vi "Init UI.vi"(8 "error in (no error)":errorcluster, 11 "HistorianCharting in":refnum<class "HistorianCharting.lvclass">) -> (0 "error out":errorcluster, 3 "HistorianCharting out":refnum<class "HistorianCharting.lvclass">)   [LabVIEW 2020, in "VolatusGUIElements.lvlib" / "HistorianCharting.lvclass"]
uses:
  HistorianCharting.lvclass
  HistorianCharting.lvclass/HistorianCharting.ctl
  <vilib>/dlg_ctls.llb/Space Constant.vi
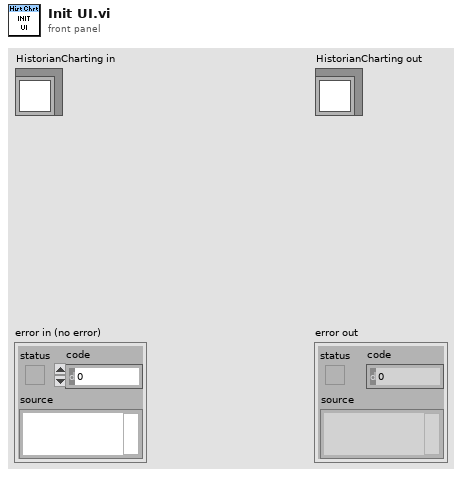
[diagram p1: front panel]
types:
  T1 = cluster{"Channel":string, "Value":dbl, "Color":u32, "Scale":bool, "Visible":bool}[]
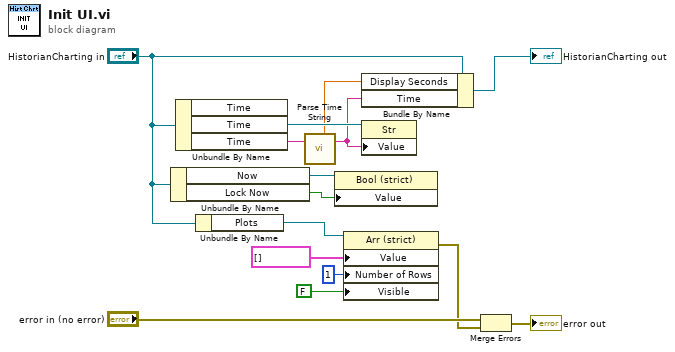
[diagram p0: block diagram]
diagram:
  n1 = Unbundle By Name("HistorianCharting in") -> ("Now"=w7:refnum<vi>, "Lock Now"=w8:bool)
  n2 = Unbundle By Name("HistorianCharting in") -> ("Time"=w5:refnum<vi>, "Time"=w3:string)  [unwired: 1 out]
  n3 = Unbundle By Name("HistorianCharting in") -> ("Plots"=w14:refnum<vi>)
  n4 = call "Parse Time String.vi"("Time String"=w3) -> ("Seconds"=w1:dbl, "Normalized String"=w2:string)  [unwired: 5 in]
  n5 = property class="Bool (strict)"(reference=w7, "Value"=w8) -> ()  [unwired: 1 in, 2 out]
  n6 = property class="Arr (strict)"(reference=w14, "Value"=T1 [], "Number of Rows"=u32 1, "Visible"=FALSE) -> (error out=w9:errorcluster)  [unwired: 1 in, 1 out]
  n7 = Bundle By Name(cluster="HistorianCharting in", "Display Seconds"=w1, "Time"=w2) -> (→"HistorianCharting out":refnum<class "HistorianCharting.lvclass">)
  n8 = property class="Str"(reference=w5, "Value"=w2) -> ()  [unwired: 1 in, 2 out]
  n9 = Merge Errors("error in (no error)", w9) -> (→"error out":errorcluster)
